vi "Initialize_Base64_URL_Encoding.vi"(7 "marshal-raw-string":bool) -> (3 "Base64 URL Encoding":refnum<class "Serializer.Base64.lvclass">)   [LabVIEW 2013, in "Serializer.Base64.lvclass"]
uses:
  Serializer.Base64.lvclass
  Serializer.Base64.lvclass/Serializer.Base64.ctl
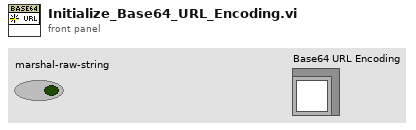
[diagram p1: front panel]
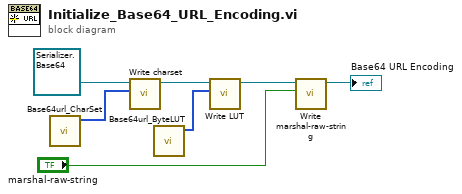
[diagram p0: block diagram]
diagram:
  n1 = call "Base64url_CharSet.vi"() -> ("base64 URL charset"=w6:u8[])  [unwired: 11 in]
  n2 = call "Write charset.vi"("charset"=w6, "Serializer.Base64 in"=refnum<class "Serializer.Base64.lvclass"> refnum ("Serializer.Base64.lvclass")) -> ("Serializer.Base64 out"=w3:refnum<class "Serializer.Base64.lvclass">)  [unwired: 8 in, 1 out]
  n3 = call "Base64url_ByteLUT.vi"() -> ("Base64 URL LUT"=w1:u32[])  [unwired: 11 in]
  n4 = call "Write LUT.vi"("LUT"=w1, "Serializer.Base64 in"=w3) -> ("Serializer.Base64 out"=w2:refnum<class "Serializer.Base64.lvclass">)  [unwired: 8 in, 1 out]
  n5 = call "Write marshal-raw-string.vi"("marshall-raw-string"="marshal-raw-string", "Serializer.Base64 in"=w2) -> ("Serializer.Base64 out"=→"Base64 URL Encoding":refnum<class "Serializer.Base64.lvclass">)  [unwired: 8 in, 1 out]
